vi "Write Measurement Preset (for N9020A).vi"(8 "error in (no error)":errorcluster, 10 "Measurement Preset":T1, 11 "Keysight 9020A in":refnum<class "Keysight 9020A.lvclass">) -> (0 "error out":errorcluster, 3 "Keysight 9020A out":refnum<class "Keysight 9020A.lvclass">)   [LabVIEW 2023, in "Spectrum Analyzer.lvlib" / "Keysight 9020A.lvclass"]
uses:
  Keysight 9020A.lvclass
  Keysight 9020A.lvclass/Keysight 9020A.ctl
  TYPE DEFINITION/Keysight 9020A/TYPE Measurement Preset.ctl
  Spectrum Analyzer.lvlib
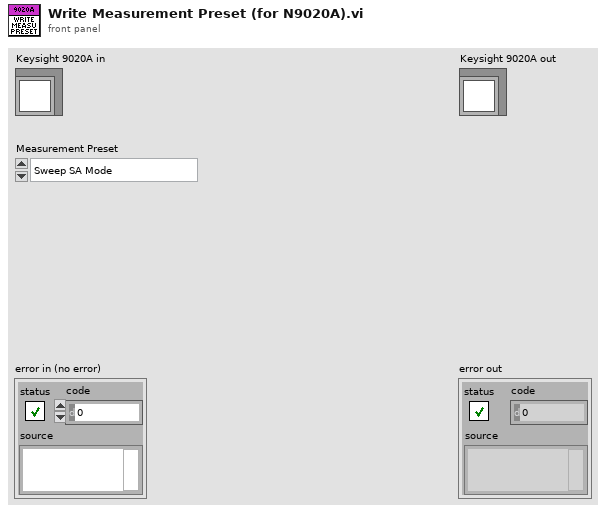
[diagram p1: front panel]
types:
  T1 = typedef "Spectrum Analyzer.lvlib/TYPE Measurement Preset.ctl" = enum16{"Sweep SA Mode", "Channel Power", "Occupied BW", "ACP", "Spurious Emission", "Spurious Emission Mask", "Burst Power (Transmit Power)"}
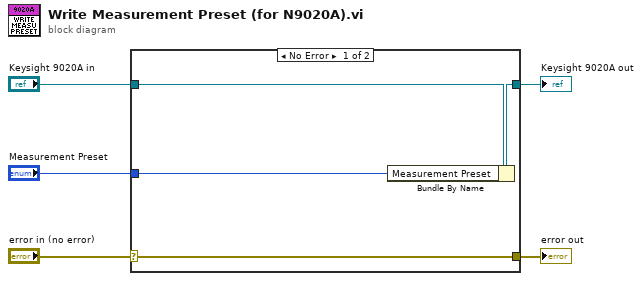
[diagram p0: block diagram]
diagram:
  n1 = case shown="No Error" "error in (no error)" {
    selector: "error in (no error)" -> [w9 w10]
    tunnel: [w9 w10] -> w4
    tunnel: [w7 w11] -> w2
    tunnel: "Keysight 9020A in" -> [w8 w11]
    tunnel: "Measurement Preset" -> [w6 _]
    frame No Error {
      n2 = Bundle By Name(cluster=w8, "Measurement Preset"=w6) -> (w7:refnum<class "Keysight 9020A.lvclass">)
    }
    frame Error {
    }
  }
  "error out" <- w4
  "Keysight 9020A out" <- w2
